vi "LV_DrawLine.vi"(8 "Connected":bool=TRUE, 9 "Phase":i32, 10 "Snapshot":T1) -> (1 "Line Picture":picture)   [LabVIEW 2018]
doc: "Use this template to build a VI to use as a subVI."
uses:
  LV_Snapshot.ctl
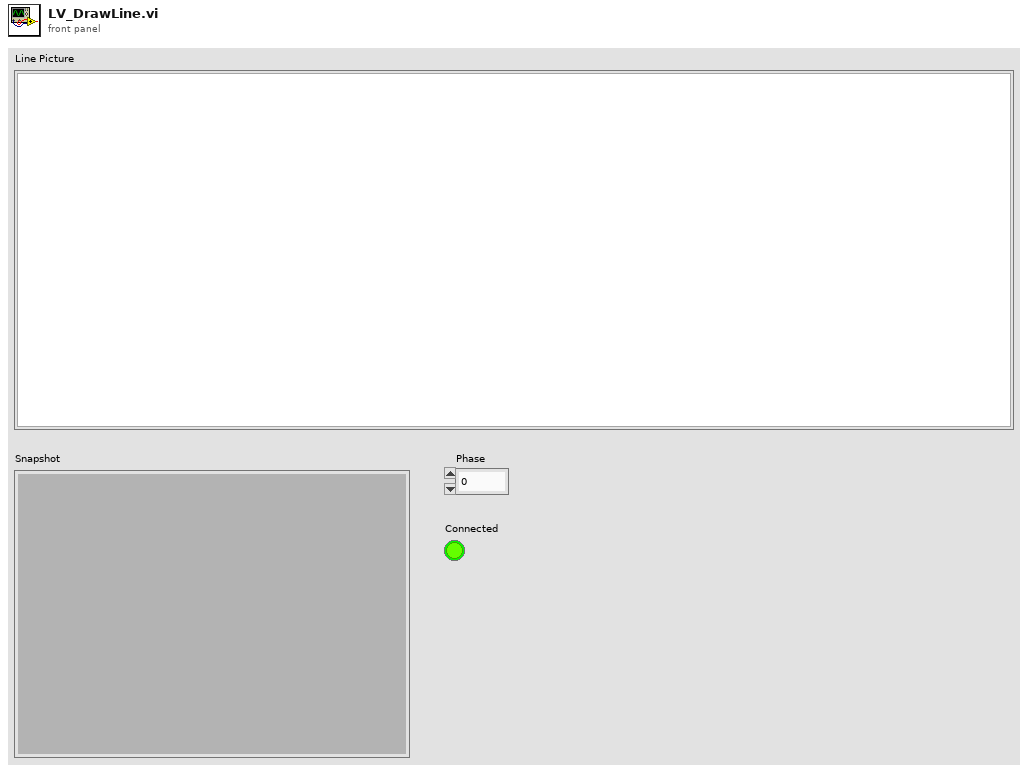
[diagram p1: front panel]
types:
  T1 = typedef "LV_Snapshot.ctl" = cluster{"DI":bool[], "DO":bool[], "IR":u16[], "Speed":u16}
  T2 = cluster{"left":i16, "top":i16, "right":i16, "bottom":i16}
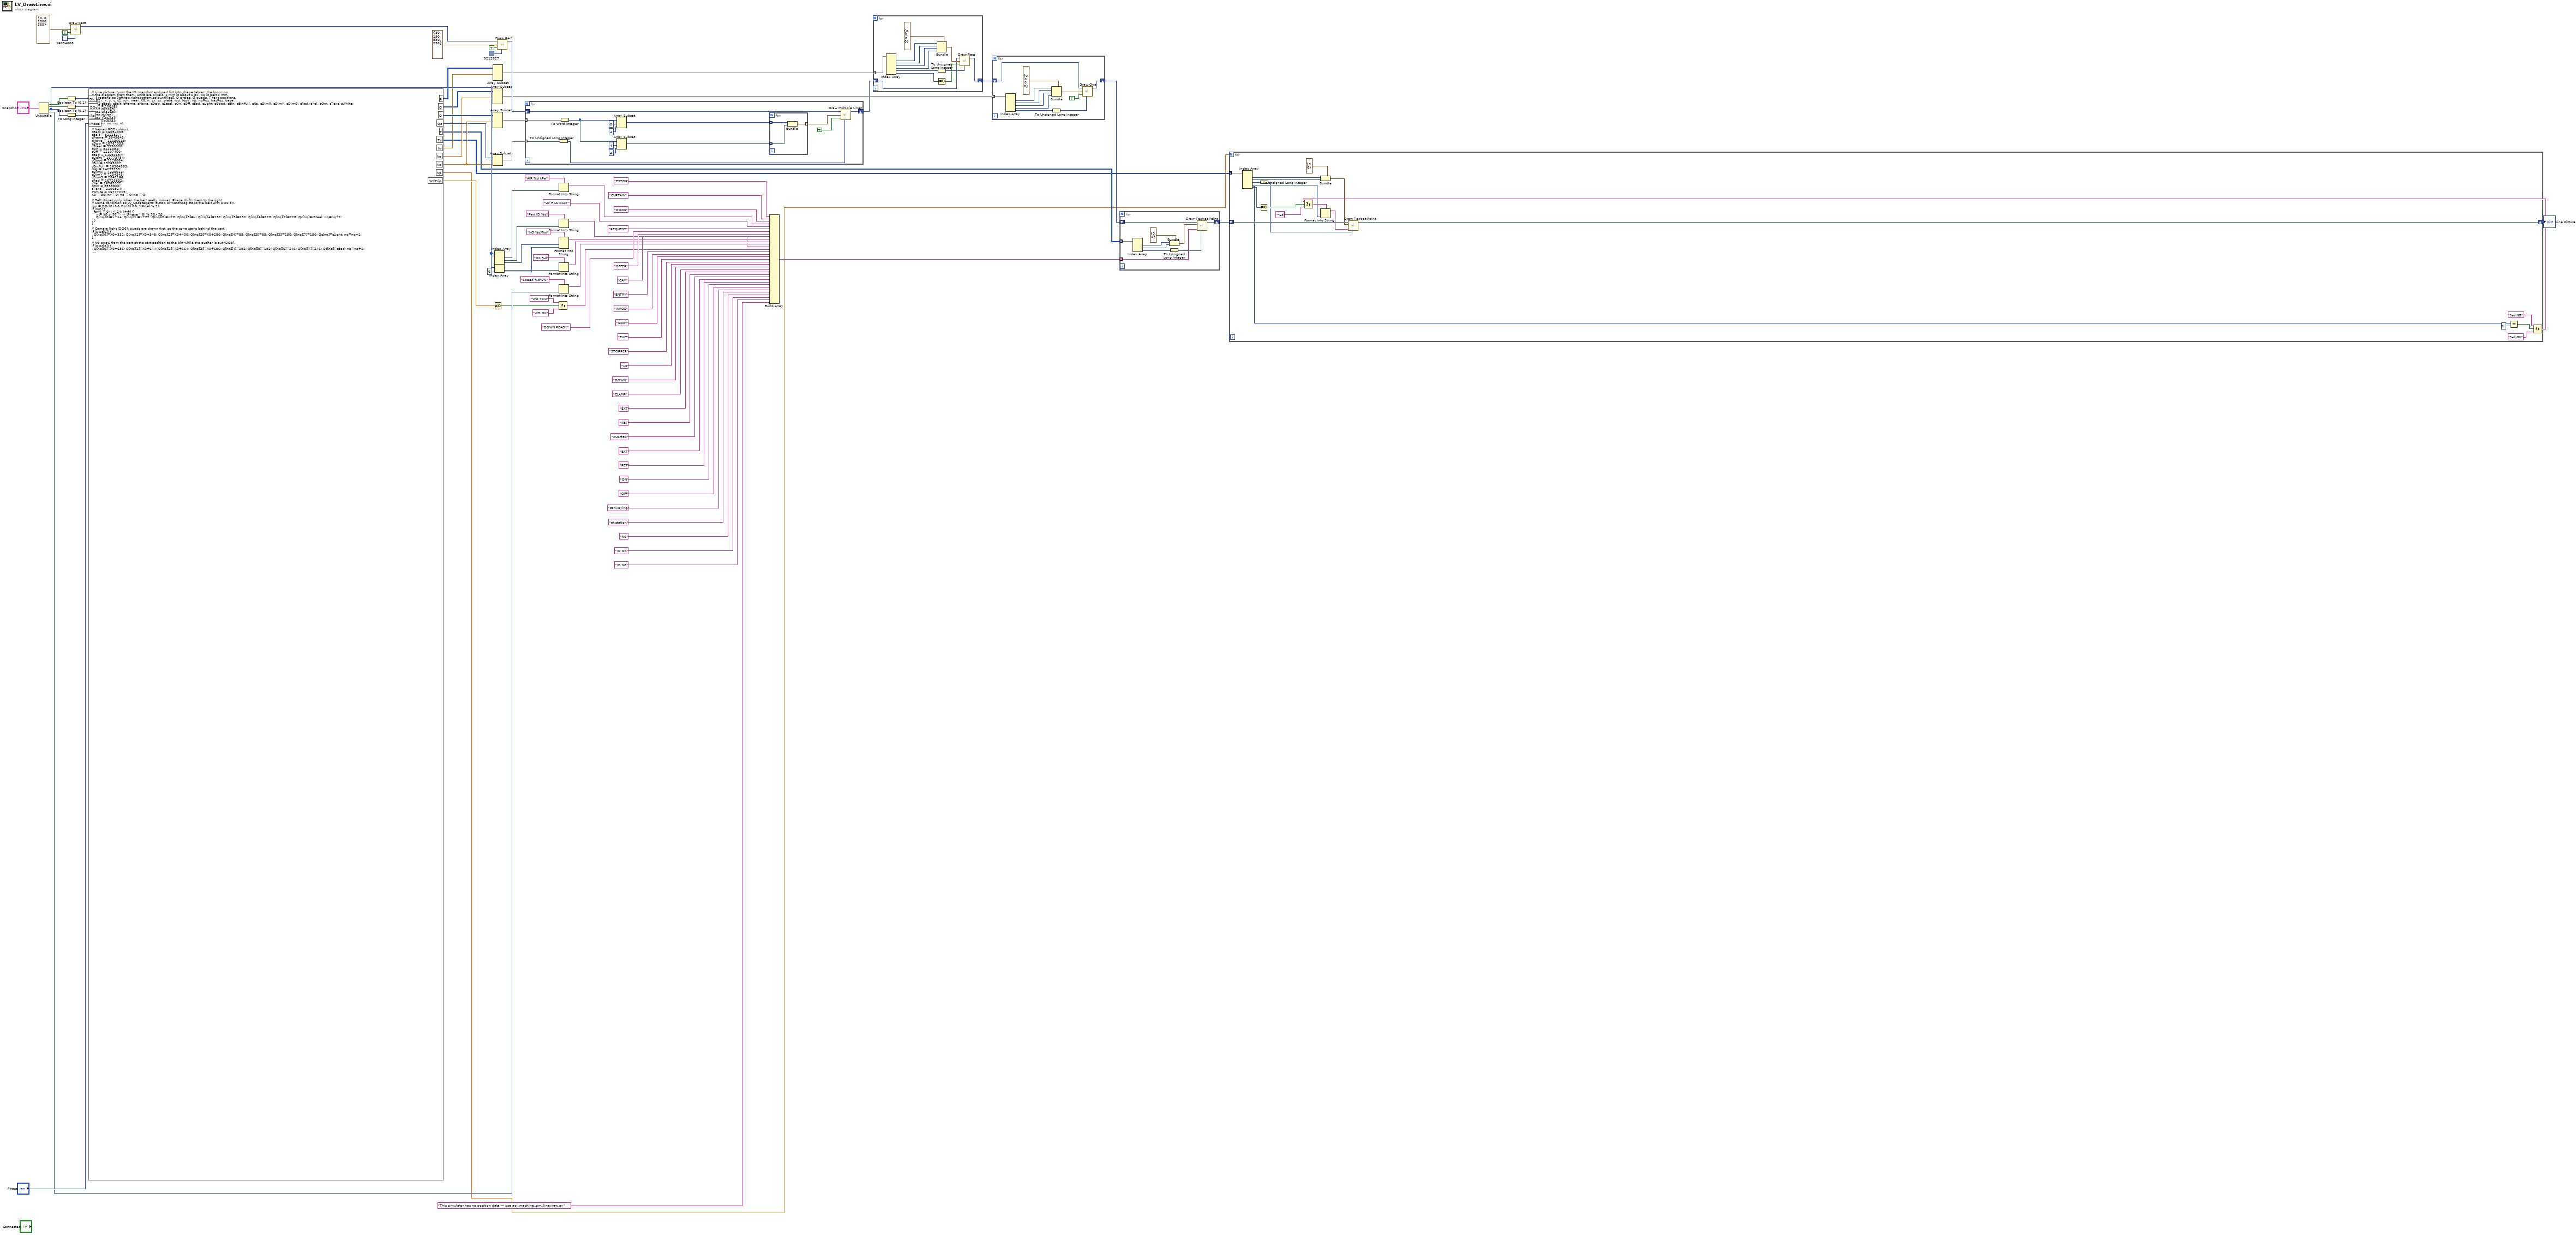
[diagram p0: block diagram]
diagram:
  n1 = Unbundle("Snapshot") -> ("DI"=w86:bool[], "DO"=w84:bool[], "IR"=w82:u16[], "Speed"=w51:u16)
  n2 = Boolean To (0,1)(Boolean=w86) -> (0, 1=w85:i16[])
  n3 = Boolean To (0,1)(Boolean=w84) -> (0, 1=w83:i16[])
  n4 = To Long Integer(number=w82) -> (32bit integer=w81:i32[])
  n5 = call <vilib>:"Draw Rect.vi"("rect"=T2 {"left"=0, "top"=0, "right"=1000, "bottom"=360}, "fill?(F)"=TRUE, "color(black)"=u32 16054008) -> ("new picture"=w76:picture)  [unwired: 6 in]
  n6 = formula code="// Line picture: turns the IO snapshot and part list into shape tables; the loops on\n// the diagram draw them. Units are pixels, 1 mm is about 1 px, X0 is belt 0 mm.\n// R rectangles [left,top,right,bottom,colour,filled], O circles, Q quads, T text positions.\nint32 i, x, y, c, c1, run, near, X0, n, sx, sy, plate, rod, topY, np, noPos, hasPos, base;\nint32 cBack, cBelt, cFrame, cMove, cStop, cSteel, cOn, cOff, cBad, cLight, cGood, cBin, cBinFull, cNg, cDimR, cDimY, cDimG, cRed, cYel, cGrn, cText, cWhite;\nint32 R[100][6];\nint32 O[20][5];\nint32 Q[32][8];\nint32 Qc[32];\nint32 T[36][3];\nint32 Tp[8][5];\nint32 nr, no, nq, nt;\n\n// Named RGB colours.\ncBack = 16054008;\ncBelt = 9212827;\ncFrame = 3949645;\ncMove = 11130613;\ncStop = 16767053;\ncSteel = 5990000;\ncOn = 3126084;\ncOff = 12107460;\ncBad = 14692657;\ncLight = 16773754;\ncGood = 3126084;\ncBin = 15265007;\ncBinFull = 16304585;\ncNg = 14239759;\ncDimR = 7220011;\ncDimY = 7234343;\ncDimG = 2842166;\ncRed = 16726832;\ncYel = 16765952;\ncGrn = 3593820;\ncText = 2106924;\ncWhite = 16777215;\nX0 = 30; nr = 0; no = 0; nq = 0;\n\n// Belt stripes only when the belt really moves; Phase shifts them to the right.\n// Same condition as LV_UpdateParts: E-stop or watchdog stops the belt with DO0 on.\nrun = DOc[0] && DIc[0] && !(IRc[4] % 2);\nif (run) {\n  for (i = 0; i < 24; i++) {\n    x = X0 + 38 * i + (Phase * 6) % 38 - 20;\n    Q[nq][0]=x+14; Q[nq][1]=x+22; Q[nq][2]=x+8; Q[nq][3]=x; Q[nq][4]=192; Q[nq][5]=192; Q[nq][6]=228; Q[nq][7]=228; Qc[nq]=cSteel; nq=nq+1;\n  }\n}\n\n// Camera light (DO6): quads are drawn first, so the cone stays behind the part.\nif (DOc[6]) {\n  Q[nq][0]=X0+332; Q[nq][1]=X0+348; Q[nq][2]=X0+400; Q[nq][3]=X0+280; Q[nq][4]=85; Q[nq][5]=85; Q[nq][6]=150; Q[nq][7]=150; Qc[nq]=cLight; nq=nq+1;\n}\n\n// NG arrow from the part at the sort position to the bin while the pusher is out (DO3).\nif (DOc[3]) {\n  Q[nq][0]=X0+636; Q[nq][1]=X0+644; Q[nq][2]=X0+664; Q[nq][3]=X0+656; Q[nq][4]=192; Q[nq][5]=192; Q[nq][6]=246; Q[nq][7]=246; Qc[nq]=cBad; nq=nq+1;\n  Q[nq][0]=X0+648; Q[nq][1]=X0+672; Q[nq][2]=X0+670; Q[nq][3]=X0+670; Q[nq][4]=246; Q[nq][5]=240; Q[nq][6]=260; Q[nq][7]=260; Qc[nq]=cBad; nq=nq+1;\n}\n\n// OK exit arrow.\nQ[nq][0]=X0+930; Q[nq][1]=X0+958; Q[nq][2]=X0+958; Q[nq][3]=X0+930; Q[nq][4]=195; Q[nq][5]=210; Q[nq][6]=210; Q[nq][7]=225; Qc[nq]=cGood; nq=nq+1;\nR[nr][0]=X0+903; R[nr][1]=204; R[nr][2]=X0+930; R[nr][3]=216; R[nr][4]=cGood; R[nr][5]=1; nr=nr+1;\n\n// Parts come from the simulator part table: IR16 count, then 3 registers per part\n// from IR17: id, front edge in 0.1 mm, truth (1 OK, 2 NG). 120 mm long.\n// Yellow at the station (stopper up or clamped), otherwise light blue.\n// Fewer than 41 IR values means a simulator without the table: no parts, show a note.\nhasPos = sizeOfDim(IRc, 0) >= 41;\nnoPos = sizeOfDim(IRc, 0) >= 6 && !hasPos;\nnp = 0;\nif (hasPos) np = min(IRc[16], 8);\nfor (i = 0; i < np; i++) {\n  base = 17 + 3 * i;\n  x = X0 + IRc[base + 1] / 10;\n  near = (DIc[8] || DIc[10]) && IRc[base + 1] >= 3920 && IRc[base + 1] <= 4050;\n  if (near) c = cStop; else c = cMove;\n  R[nr][0]=x-120; R[nr][1]=150; R[nr][2]=x; R[nr][3]=190; R[nr][4]=c; R[nr][5]=1; nr=nr+1;\n  R[nr][0]=x-120; R[nr][1]=150; R[nr][2]=x; R[nr][3]=190; R[nr][4]=cFrame; R[nr][5]=0; nr=nr+1;\n  Tp[i][0] = x - 112; Tp[i][1] = 162; Tp[i][3] = IRc[base];\n  if (IRc[base + 2] == 2) { Tp[i][2] = cBad; Tp[i][4] = 1; }\n  else { Tp[i][2] = cText; Tp[i][4] = 2 * IRc[base + 2]; }\n}\n\n// Stopper: DO1 raises the post above the belt. Sensors DI8 UP, DI9 DOWN.\nif (DOc[1]) topY = 165; else topY = 232;\nR[nr][0]=X0+400; R[nr][1]=topY; R[nr][2]=X0+408; R[nr][3]=252; R[nr][4]=cFrame; R[nr][5]=1; nr=nr+1;\nif (DIc[8]) c=cOn; else c=cOff; O[no][0]=X0+419-5; O[no][1]=262-5; O[no][2]=X0+419+5; O[no][3]=262+5; O[no][4]=c; no=no+1;\nif (DIc[9]) c=cOn; else c=cOff; O[no][0]=X0+459-5; O[no][1]=262-5; O[no][2]=X0+459+5; O[no][3]=262+5; O[no][4]=c; no=no+1;\n\n// Clamp: two plates; DO2 moves them 25 px inward. Sensors DI10 EXT, DI11 RET.\nif (DOc[2]) plate = 0; else plate = 25;\nR[nr][0]=X0+268-plate; R[nr][1]=118; R[nr][2]=X0+280-plate; R[nr][3]=160; R[nr][4]=cSteel; R[nr][5]=1; nr=nr+1;\nR[nr][0]=X0+400+plate; R[nr][1]=118; R[nr][2]=X0+412+plate; R[nr][3]=160; R[nr][4]=cSteel; R[nr][5]=1; nr=nr+1;\nif (DIc[10]) c=cOn; else c=cOff; O[no][0]=X0+447-5; O[no][1]=132-5; O[no][2]=X0+447+5; O[no][3]=132+5; O[no][4]=c; no=no+1;\nif (DIc[11]) c=cOn; else c=cOff; O[no][0]=X0+490-5; O[no][1]=132-5; O[no][2]=X0+490+5; O[no][3]=132+5; O[no][4]=c; no=no+1;\n\n// Camera body.\nR[nr][0]=X0+320; R[nr][1]=42; R[nr][2]=X0+362; R[nr][3]=75; R[nr][4]=cFrame; R[nr][5]=1; nr=nr+1;\nR[nr][0]=X0+332; R[nr][1]=75; R[nr][2]=X0+348; R[nr][3]=85; R[nr][4]=cSteel; R[nr][5]=1; nr=nr+1;\n\n// Pusher above the middle of a part at the sort position; DO3 extends the rod.\n// Sensors DI12 EXT, DI13 RET.\nif (DOc[3]) rod = 146; else rod = 108;\nR[nr][0]=X0+626; R[nr][1]=60; R[nr][2]=X0+654; R[nr][3]=96; R[nr][4]=cSteel; R[nr][5]=1; nr=nr+1;\nR[nr][0]=X0+636; R[nr][1]=96; R[nr][2]=X0+644; R[nr][3]=rod; R[nr][4]=cFrame; R[nr][5]=1; nr=nr+1;\nR[nr][0]=X0+620; R[nr][1]=rod; R[nr][2]=X0+660; R[nr][3]=rod+6; R[nr][4]=cFrame; R[nr][5]=1; nr=nr+1;\nif (DIc[12]) c=cOn; else c=cOff; O[no][0]=X0+667-5; O[no][1]=80-5; O[no][2]=X0+667+5; O[no][3]=80+5; O[no][4]=c; no=no+1;\nif (DIc[13]) c=cOn; else c=cOff; O[no][0]=X0+710-5; O[no][1]=80-5; O[no][2]=X0+710+5; O[no][3]=80+5; O[no][4]=c; no=no+1;\n\n// NG bin below the sort position (685..715): IR2 parts, 10 per row, red when full (DI14).\nif (DIc[14]) c = cBinFull; else c = cBin;\nR[nr][0]=X0+635; R[nr][1]=262; R[nr][2]=X0+765; R[nr][3]=340; R[nr][4]=c; R[nr][5]=1; nr=nr+1;\nR[nr][0]=X0+635; R[nr][1]=262; R[nr][2]=X0+765; R[nr][3]=340; R[nr][4]=cFrame; R[nr][5]=0; nr=nr+1;\nn = min(IRc[2], 20);\nfor (i = 0; i < n; i++) {\n  sx = X0 + 641 + 12 * (i % 10);\n  sy = 325 - 16 * ((i - i % 10) / 10);\n  R[nr][0]=sx; R[nr][1]=sy; R[nr][2]=sx+10; R[nr][3]=sy+10; R[nr][4]=cNg; R[nr][5]=1; nr=nr+1;\n}\n\n// Belt sensors DI4..7 just under the belt. INPOS sits left of the stopper post.\nif (DIc[4]) c=cOn; else c=cOff; O[no][0]=X0+40-5; O[no][1]=244-5; O[no][2]=X0+40+5; O[no][3]=244+5; O[no][4]=c; no=no+1;\nif (DIc[5]) c=cOn; else c=cOff; O[no][0]=X0+392-5; O[no][1]=244-5; O[no][2]=X0+392+5; O[no][3]=244+5; O[no][4]=c; no=no+1;\nif (DIc[6]) c=cOn; else c=cOff; O[no][0]=X0+700-5; O[no][1]=244-5; O[no][2]=X0+700+5; O[no][3]=244+5; O[no][4]=c; no=no+1;\nif (DIc[7]) c=cOn; else c=cOff; O[no][0]=X0+890-5; O[no][1]=244-5; O[no][2]=X0+890+5; O[no][3]=244+5; O[no][4]=c; no=no+1;\n\n// Light tower DO8..10.\nR[nr][0]=958; R[nr][1]=88; R[nr][2]=962; R[nr][3]=128; R[nr][4]=cSteel; R[nr][5]=1; nr=nr+1;\nif (DOc[8]) c = cRed; else c = cDimR; O[no][0]=949; O[no][1]=10; O[no][2]=971; O[no][3]=32; O[no][4]=c; no=no+1;\nif (DOc[9]) c = cYel; else c = cDimY; O[no][0]=949; O[no][1]=34; O[no][2]=971; O[no][3]=56; O[no][4]=c; no=no+1;\nif (DOc[10]) c = cGrn; else c = cDimG; O[no][0]=949; O[no][1]=58; O[no][2]=971; O[no][3]=80; O[no][4]=c; no=no+1;\n\n// Buzzer DO11: blinks with Phase.\nif (DOc[11] && (Phase % 10) < 5) {\n  Q[nq][0]=905; Q[nq][1]=925; Q[nq][2]=925; Q[nq][3]=905; Q[nq][4]=42; Q[nq][5]=28; Q[nq][6]=68; Q[nq][7]=54; Qc[nq]=cBad; nq=nq+1;\n}\n\n// Safety DI0..3: any fault turns the frame red too.\nif (DIc[0]) c=cOn; else c=cBad; R[nr][0]=10; R[nr][1]=12; R[nr][2]=10+14; R[nr][3]=12+14; R[nr][4]=c; R[nr][5]=1; nr=nr+1;\nif (DIc[1]) c=cOn; else c=cBad; R[nr][0]=10; R[nr][1]=34; R[nr][2]=10+14; R[nr][3]=34+14; R[nr][4]=c; R[nr][5]=1; nr=nr+1;\nif (DIc[2]) c=cOn; else c=cBad; R[nr][0]=10; R[nr][1]=56; R[nr][2]=10+14; R[nr][3]=56+14; R[nr][4]=c; R[nr][5]=1; nr=nr+1;\nif (DIc[3]) c=cOn; else c=cBad; R[nr][0]=10; R[nr][1]=78; R[nr][2]=10+14; R[nr][3]=78+14; R[nr][4]=c; R[nr][5]=1; nr=nr+1;\nif (DIc[0] && DIc[1] && DIc[2] && DIc[3]) c = cOff; else c = cBad;\nR[nr][0]=4; R[nr][1]=6; R[nr][2]=130; R[nr][3]=98; R[nr][4]=c; R[nr][5]=0; nr=nr+1;\n\n// Handshake: DI15 UP HAS PART, DO4 REQUEST, DI16 DOWN READY, DO5 OFFER.\nif (DIc[15]) c=cOn; else c=cOff; R[nr][0]=4; R[nr][1]=104; R[nr][2]=4+14; R[nr][3]=104+14; R[nr][4]=c; R[nr][5]=1; nr=nr+1;\nif (DOc[4]) c=cOn; else c=cOff; R[nr][0]=4; R[nr][1]=122; R[nr][2]=4+14; R[nr][3]=122+14; R[nr][4]=c; R[nr][5]=1; nr=nr+1;\nif (DIc[16]) c=cOn; else c=cOff; R[nr][0]=845; R[nr][1]=104; R[nr][2]=845+14; R[nr][3]=104+14; R[nr][4]=c; R[nr][5]=1; nr=nr+1;\nif (DOc[5]) c=cOn; else c=cOff; R[nr][0]=845; R[nr][1]=122; R[nr][2]=845+14; R[nr][3]=122+14; R[nr][4]=c; R[nr][5]=1; nr=nr+1;\n\n// Legend.\nR[nr][0]=815; R[nr][1]=262; R[nr][2]=960; R[nr][3]=346; R[nr][4]=cOff; R[nr][5]=0; nr=nr+1;\nO[no][0]=822; O[no][1]=270; O[no][2]=832; O[no][3]=280; O[no][4]=cOn; no=no+1;\nO[no][0]=880; O[no][1]=270; O[no][2]=890; O[no][3]=280; O[no][4]=cOff; no=no+1;\nR[nr][0]=822; R[nr][1]=291; R[nr][2]=840; R[nr][3]=303; R[nr][4]=cMove; R[nr][5]=1; nr=nr+1;\nR[nr][0]=822; R[nr][1]=291; R[nr][2]=840; R[nr][3]=303; R[nr][4]=cFrame; R[nr][5]=0; nr=nr+1;\nR[nr][0]=822; R[nr][1]=311; R[nr][2]=840; R[nr][3]=323; R[nr][4]=cStop; R[nr][5]=1; nr=nr+1;\nR[nr][0]=822; R[nr][1]=311; R[nr][2]=840; R[nr][3]=323; R[nr][4]=cFrame; R[nr][5]=0; nr=nr+1;\n\n// Text positions and colours, same order as the string array on the diagram.\nif (IRc[4] % 2) c1 = cBad; else c1 = cGood;\nWdTrip = IRc[4] % 2;\nnt = 0;\nx=30; y=12; T[nt][0]=x; T[nt][1]=y; T[nt][2]=cText; nt=nt+1;\nx=30; y=34; T[nt][0]=x; T[nt][1]=y; T[nt][2]=cText; nt=nt+1;\nx=30; y=56; T[nt][0]=x; T[nt][1]=y; T[nt][2]=cText; nt=nt+1;\nx=30; y=78; T[nt][0]=x; T[nt][1]=y; T[nt][2]=cText; nt=nt+1;\nx=22; y=103; T[nt][0]=x; T[nt][1]=y; T[nt][2]=cText; nt=nt+1;\nx=22; y=121; T[nt][0]=x; T[nt][1]=y; T[nt][2]=cText; nt=nt+1;\nx=863; y=103; T[nt][0]=x; T[nt][1]=y; T[nt][2]=cText; nt=nt+1;\nx=863; y=121; T[nt][0]=x; T[nt][1]=y; T[nt][2]=cText; nt=nt+1;\nx=X0+328; y=50; T[nt][0]=x; T[nt][1]=y; T[nt][2]=cWhite; nt=nt+1;\nx=X0+641; y=267; T[nt][0]=x; T[nt][1]=y; T[nt][2]=cText; nt=nt+1;\nx=X0+906; y=176; T[nt][0]=x; T[nt][1]=y; T[nt][2]=cText; nt=nt+1;\nx=10; y=338; T[nt][0]=x; T[nt][1]=y; T[nt][2]=cText; nt=nt+1;\nx=120; y=338; T[nt][0]=x; T[nt][1]=y; T[nt][2]=cText; nt=nt+1;\nx=250; y=338; T[nt][0]=x; T[nt][1]=y; T[nt][2]=c1; nt=nt+1;\nx=X0+49; y=237; T[nt][0]=x; T[nt][1]=y; T[nt][2]=cText; nt=nt+1;\nx=X0+342; y=237; T[nt][0]=x; T[nt][1]=y; T[nt][2]=cText; nt=nt+1;\nx=X0+709; y=237; T[nt][0]=x; T[nt][1]=y; T[nt][2]=cText; nt=nt+1;\nx=X0+899; y=237; T[nt][0]=x; T[nt][1]=y; T[nt][2]=cText; nt=nt+1;\nx=X0+414; y=236; T[nt][0]=x; T[nt][1]=y; T[nt][2]=cText; nt=nt+1;\nx=X0+427; y=255; T[nt][0]=x; T[nt][1]=y; T[nt][2]=cText; nt=nt+1;\nx=X0+467; y=255; T[nt][0]=x; T[nt][1]=y; T[nt][2]=cText; nt=nt+1;\nx=X0+442; y=104; T[nt][0]=x; T[nt][1]=y; T[nt][2]=cText; nt=nt+1;\nx=X0+455; y=125; T[nt][0]=x; T[nt][1]=y; T[nt][2]=cText; nt=nt+1;\nx=X0+498; y=125; T[nt][0]=x; T[nt][1]=y; T[nt][2]=cText; nt=nt+1;\nx=X0+662; y=52; T[nt][0]=x; T[nt][1]=y; T[nt][2]=cText; nt=nt+1;\nx=X0+675; y=73; T[nt][0]=x; T[nt][1]=y; T[nt][2]=cText; nt=nt+1;\nx=X0+718; y=73; T[nt][0]=x; T[nt][1]=y; T[nt][2]=cText; nt=nt+1;\nx=834; y=268; T[nt][0]=x; T[nt][1]=y; T[nt][2]=cText; nt=nt+1;\nx=892; y=268; T[nt][0]=x; T[nt][1]=y; T[nt][2]=cText; nt=nt+1;\nx=846; y=288; T[nt][0]=x; T[nt][1]=y; T[nt][2]=cText; nt=nt+1;\nx=846; y=308; T[nt][0]=x; T[nt][1]=y; T[nt][2]=cText; nt=nt+1;\nif (DOc[3]) x=X0+622; else x=-200; y=237; T[nt][0]=x; T[nt][1]=y; T[nt][2]=cBad; nt=nt+1;\nx=822; y=328; T[nt][0]=x; T[nt][1]=y; T[nt][2]=cText; nt=nt+1;\nx=880; y=328; T[nt][0]=x; T[nt][1]=y; T[nt][2]=cBad; nt=nt+1;\nif (noPos) x=250; else x=-2000; y=160; T[nt][0]=x; T[nt][1]=y; T[nt][2]=cBad; nt=nt+1;\nNr = nr; No = no; Nq = nq; Np = np;"("DIc"=w85, "DOc"=w83, "IRc"=w81, "Phase"="Phase") -> ("R"=w66:i32[][], "O"=w62:i32[][], "Q"=w72:i32[][], "Qc"=w70:i32[], "T"=w7:i32[][], "Tp"=w4:i32[][], "Nr"=w65:dbl, "No"=w61:dbl, "Nq"=w71:dbl, "Np"=w6:dbl, "WdTrip"=w48:dbl)
  n7 = Array Subset(array=w70, length=w71) -> (w68:i32[])  [unwired: 1 in]
  n8 = Array Subset(array=w66, length (row)=w65) -> (w63:i32[][])  [unwired: 3 in]
  n9 = Array Subset(array=w62, length (row)=w61) -> (w59:i32[][])  [unwired: 3 in]
  n10 = Array Subset(array=w72, length (row)=w71) -> (w67:i32[][])  [unwired: 3 in]
  n11 = Not Equal To 0?(x=w48) -> (x != 0?=w46:bool)
  n12 = Index Array(array=w82) -> (element #1=w57:u16, element #2=w49:u16, element #3=w55:u16, element #6=w53:u16)  [unwired: 6 in, 2 out]
  n13 = Index Array(array=w82, index=6) -> (element=w1:u16)
  n14 = call <vilib>:"Draw Rect.vi"("picture"=w76, "rect"=T2 {"left"=30, "top"=190, "right"=930, "bottom"=230}, "fill?(F)"=TRUE, "color(black)"=u32 9212827) -> ("new picture"=w69:picture)  [unwired: 5 in]
  n15 = for {
    shift-right: [w100] -> w64
    shift-left: w69 -> [w101]
    tunnel: w68 -> [w98] mode=indexing
    tunnel: w67 -> [w96] mode=indexing
    n16 = To Unsigned Long Integer(number=w98) -> (unsigned 32bit integer=w97:u32)
    n17 = To Word Integer(number=w96) -> (16bit integer=w95:i16[])
    n18 = Array Subset(array=w95, index=0, length=4) -> (w90:i16[])
    n19 = Array Subset(array=w95, index=4, length=4) -> (w89:i16[])
    n20 = for {
      tunnel: w90 -> [w104] mode=indexing
      tunnel: w89 -> [w103] mode=indexing
      tunnel: [w102] -> w88 mode=indexing
      n21 = Bundle(w104, w103) -> (w102:cluster{i16, i16})  [unwired: 1 in]
    }
    n22 = call <vilib>:"Draw Multiple Lines.vi"("picture"=w101, "line endpoints"=w88, "fill?(F)"=TRUE, "color(black)"=w97) -> ("new picture"=w100:picture)  [unwired: 5 in]
  }
  n23 = Select(t="WD TRIP", s=w46, f="WD OK") -> (s? t:f=w31:string)
  n24 = Format Into String(format string="AIR %d kPa", w57) -> (resulting string=w41:string)  [unwired: 2 in, 1 out]
  n25 = Format Into String(format string="Part ID %d", w49) -> (resulting string=w32:string)  [unwired: 2 in, 1 out]
  n26 = Format Into String(format string="NG %d/%d", w55, w1) -> (resulting string=w35:string)  [unwired: 2 in, 1 out]
  n27 = Format Into String(format string="OK %d", w53) -> (resulting string=w34:string)  [unwired: 2 in, 1 out]
  n28 = Format Into String(format string="Speed %d%%", w51) -> (resulting string=w33:string)  [unwired: 2 in, 1 out]
  n29 = Build Array("ESTOP", "CURTAIN", "DOOR", w41, "UP HAS PART", "REQUEST", "DOWN READY", "OFFER", "CAM", w35, w34, w33, w32, w31, "ENTRY", "INPOS", "SORT", "EXIT", "STOPPER", "UP", "DOWN", "CLAMP", "EXT", "RET", "PUSHER", "EXT", "RET", "ON", "OFF", "conveying", "at station", "NG", "ID OK", "ID NG", "This simulator has no position data — use aoi_machine_sim_lineview.py") -> (w8:string[])
  n30 = for {
    shift-right: [w109] -> w60
    shift-left: w64 -> [w110]
    tunnel: w63 -> [w117] mode=indexing
    n31 = Index Array(array=w117) -> (element #1=w115:i32, element #2=w114:i32, element #3=w113:i32, element #4=w112:i32, element #5=w108:i32, element #6=w106:i32)  [unwired: 6 in]
    n32 = To Unsigned Long Integer(number=w108) -> (unsigned 32bit integer=w107:u32)
    n33 = Not Equal To 0?(x=w106) -> (x != 0?=w105:bool)
    n34 = Bundle(cluster=T2 {"left"=0, "top"=0, "right"=0, "bottom"=0} ("rect"), "left"=w115, "top"=w114, "right"=w113, "bottom"=w112) -> (w111:T2)
    n35 = call <vilib>:"Draw Rect.vi"("picture"=w110, "rect"=w111, "fill?(F)"=w105, "color(black)"=w107) -> ("new picture"=w109:picture)  [unwired: 5 in]
  }
  n36 = for {
    shift-right: [w121] -> w9
    shift-left: w60 -> [w122]
    tunnel: w59 -> [w129] mode=indexing
    n37 = Index Array(array=w129) -> (element #1=w127:i32, element #2=w126:i32, element #3=w125:i32, element #4=w124:i32, element #5=w120:i32)  [unwired: 5 in]
    n38 = To Unsigned Long Integer(number=w120) -> (unsigned 32bit integer=w119:u32)
    n39 = Bundle(cluster=T2 {"left"=0, "top"=0, "right"=0, "bottom"=0} ("rect"), "left"=w127, "top"=w126, "right"=w125, "bottom"=w124) -> (w123:T2)
    n40 = call <vilib>:"Draw Oval.vi"("picture"=w122, "rect"=w123, "fill?(F)"=TRUE, "color(black)"=w119) -> ("new picture"=w121:picture)  [unwired: 5 in]
  }
  n41 = for {
    shift-right: [w138] -> w5
    shift-left: w9 -> [w139]
    tunnel: w8 -> [w137] mode=indexing
    tunnel: w7 -> [w136] mode=indexing
    n42 = Index Array(array=w136) -> (element #1=w134:i32, element #2=w133:i32, element #3=w131:i32)  [unwired: 3 in]
    n43 = To Unsigned Long Integer(number=w131) -> (unsigned 32bit integer=w130:u32)
    n44 = Bundle(cluster=cluster{"x":i16, "y":i16} {"x"=0, "y"=0} ("origin"), "x"=w134, "y"=w133) -> (w132:cluster{"x":i16, "y":i16})
    n45 = call <vilib>:"Draw Text at Point.vi"("text color(black)"=w130, "text"=w137, "origin"=w132, "picture"=w139) -> ("new picture"=w138:picture)  [unwired: 6 in, 1 out]
  }
  n46 = for {
    N: w6 -> [_]
    shift-right: [w158] -> w3
    shift-left: w5 -> [w159]
    tunnel: w4 -> [w157] mode=indexing
    n47 = Index Array(array=w157) -> (element #1=w149:i32, element #2=w148:i32, element #3=w146:i32, element #4=w152:i32, element #5=w156:i32)  [unwired: 5 in]
    n48 = To Unsigned Long Integer(number=w146) -> (unsigned 32bit integer=w145:u32)
    n49 = Not Equal To 0?(x=w156) -> (x != 0?=w155:bool)
    n50 = Bundle(cluster=cluster{"x":i16, "y":i16} {"x"=0, "y"=0} ("origin"), "x"=w149, "y"=w148) -> (w147:cluster{"x":i16, "y":i16})
    n51 = Equal?(x=w156, y=1) -> (x = y?=w143:bool)
    n52 = Select(t="%d NG", s=w143, f="%d OK") -> (s? t:f=w140:string)
    n53 = Select(t=w140, s=w155, f="%d") -> (s? t:f=w153:string)
    n54 = Format Into String(format string=w153, w152) -> (resulting string=w151:string)  [unwired: 2 in, 1 out]
    n55 = call <vilib>:"Draw Text at Point.vi"("text color(black)"=w145, "text"=w151, "origin"=w147, "picture"=w159) -> ("new picture"=w158:picture)  [unwired: 6 in, 1 out]
  }
  "Line Picture" <- w3
